vi "Update Pin Map from XML.vi"(8 "error in":errorcluster, 11 "request data":T2) -> (0 "error out":errorcluster, 3 "response data":T1)   [LabVIEW 2021, in "NI Pin Map V1 Client.lvlib"]
uses:
  NI Pin Map V1 Client.lvlib
  gRPC/Generated APIs/ni/measurementlink/pinmap/v1/RPC Messages/ni_measurementlink_pinmap_v1_UpdatePinMapFromXmlRequest.ctl
  gRPC/Generated APIs/ni/measurementlink/pinmap/v1/RPC Messages/ni_measurementlink_pinmap_v1_PinMap.ctl
  Discovery V1/TypeDefs/gRPC Client Cache FGV Action.ctl
  gRPC/Generated APIs/ni/measurementlink/pinmap/v1/ni.measurementlink.pinmap.v1.api.lvlib
  Discovery V1/NI Discovery V1 Client.lvlib
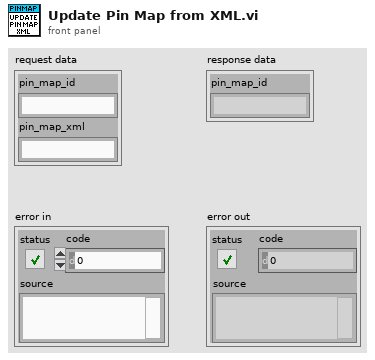
[diagram p1: front panel]
types:
  T1 = typedef "ni.measurementlink.pinmap.v1.api.lvlib/ni_measurementlink_pinmap_v1_PinMap.ctl" = cluster{"pin_map_id":string}
  T2 = typedef "ni.measurementlink.pinmap.v1.api.lvlib/ni_measurementlink_pinmap_v1_UpdatePinMapFromXmlRequest.ctl" = cluster{"pin_map_id":string, "pin_map_xml":string}
  T3 = typedef "NI Discovery V1 Client.lvlib/gRPC Client Cache FGV Action.ctl" = enum16{"Get Client", "Recreate Client", "Destroy Client", "Update ClusterId"}
  T4 = typedef "grpc-lvsupport-release.lvlib/grpcId.ctl" = u64
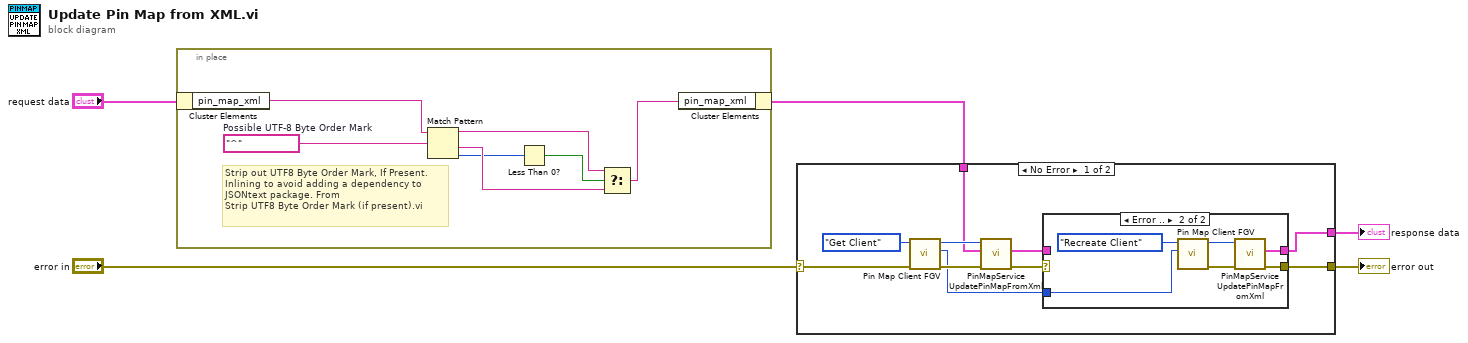
[diagram p0: block diagram]
diagram:
  n1 = in-place {
    w8 = "^﻿"  # Possible UTF-8 Byte Order Mark
    # "Strip out UTF8 Byte Order Mark, If Present.\nInlining to avoid adding a dependency to\nJSONtext package. From\nStrip UTF8 Byte Order Mark (if present).vi"
    n2 = in-place-cluster #1("request data") -> ("pin_map_xml"=w7:string)
    n3 = Match Pattern(string=w7, regular expression=w8) -> (before substring=w10:string, after substring=w12:string, offset past match=w9:i32)  [unwired: 1 in, 1 out]
    n4 = Less Than 0?(x=w9) -> (x < 0?=w11:bool)
    n5 = Select(t=w10, s=w11, f=w12) -> (s? t:f=w6:string)
    n6 = in-place-cluster #1("pin_map_xml"=w6) -> (w1:T2)
  }
  n7 = case shown="No Error" "error in" {
    selector: "error in" -> [w22 w31]
    tunnel: [w18 w31] -> w4
    tunnel: [w16 _] -> w3
    tunnel: w1 -> [w13 _]
    frame No Error {
      n8 = call "Pin Map Client FGV.vi"("error in"=w22, "action"=gRPC_Client_Cache_FGV_Action."Get Client") -> ("error out"=w21:errorcluster, "unique id out"=w14:u64, "grpc client id"=w20:T4)  [unwired: 7 in]
      n9 = call "PinMapService UpdatePinMapFromXml.vi"("error in"=w21, "Request Data"=w13, "gRPC ID"=w20) -> ("error out"=w19:errorcluster, "Response Data"=w15:T1)  [unwired: 6 in, 1 out]
      n10 = case shown="Error .." w19 {
        selector: w19 -> [w24 _]
        tunnel: [w24 w27] -> w18
        tunnel: [w23 w26] -> w16
        tunnel: w15 -> [w23 _]
        tunnel: w14 -> [_ w25]
        frame No Error {
        }
        frame Error {
          n11 = call "Pin Map Client FGV.vi"("unique id in"=w25, "action"=gRPC_Client_Cache_FGV_Action."Recreate Client") -> ("error out"=w28:errorcluster, "grpc client id"=w29:T4)  [unwired: 7 in, 1 out]
          n12 = call "PinMapService UpdatePinMapFromXml.vi"("error in"=w28, "gRPC ID"=w29) -> ("error out"=w27:errorcluster, "Response Data"=w26:T1)  [unwired: 7 in, 1 out]
        }
      }
    }
    frame Error {
    }
  }
  "error out" <- w4
  "response data" <- w3
